vi "RemoteVI Loop Flags.vi"(0 "clients":T1(array[cluster]), 5 "last geometry":u32, 7 "last click":u32, 9 "popup was open?":bool) -> (4 "now":u32, 6 "look?":bool, 8 "geometry due?":bool, 10 "remote click?":bool, 15 "recent click?":bool)   [LabVIEW 2020, in "RemoteVI.lvlib"]
doc: "The timing decisions at the start of a server loop iteration: now (tick count ms); geometry due? when 500 ms have passed since last geometry; look? (list the popups) when a client is connected, the geometry is due or a popup was open last time; remote click? within 1 s and recent click? within 300 ms after a client last posted a message that may open a popup (last click). Pure apart from reading the tick count."
uses:
  RemoteVI.lvlib
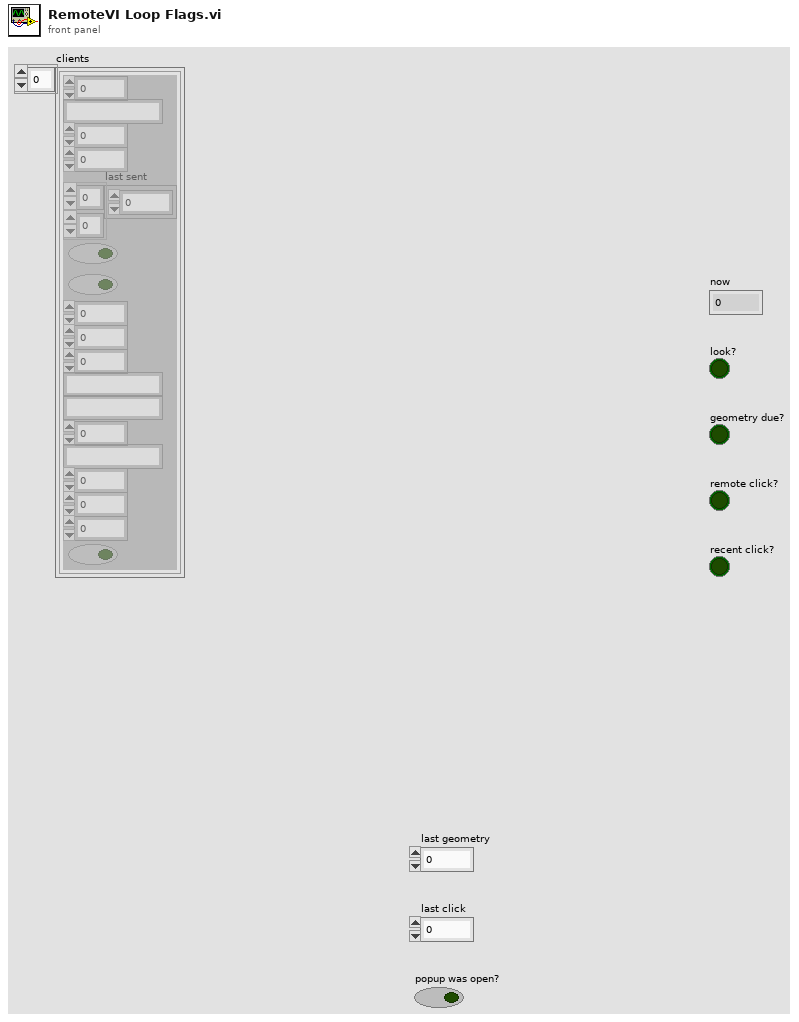
[diagram p1: front panel]
types:
  T1 = cluster{"connection":u32, "rx buffer":string, "seq":u32, "acked":u32, "last sent":u32[][], "tracking":bool, "closed":bool, "mods":u8, "mods set":u8, "popup since":u32, "windows sent":string, "window frames":cluster{"id":u64, "pixels":u32[][]}[], "key window":u64, "address":string, "since":dbl, "last input":dbl, "bytes":dbl, "view only":bool}[]
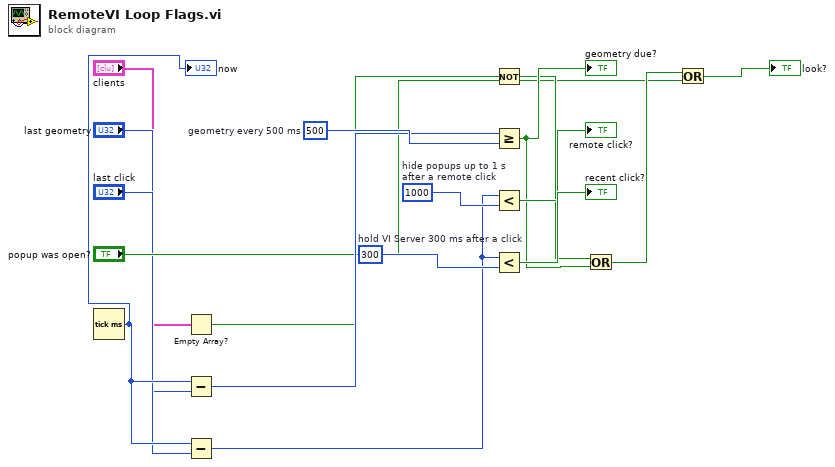
[diagram p0: block diagram]
diagram:
  w16 = u32 300  # hold VI Server 300 ms after a click
  w14 = u32 1000  # hide popups up to 1 s after a remote click
  w9 = u32 500  # geometry every 500 ms
  n1 = Tick Count (ms)() -> (millisecond timer value=w5:u32)
  "now" <- w5
  n2 = Empty Array?(array="clients") -> (empty?=w6:bool)
  n3 = Subtract(x=w5, y="last geometry") -> (x-y=w8:u32)
  n4 = Subtract(x=w5, y="last click") -> (x-y=w13:u32)
  n5 = Not(x=w6) -> (.not. x?=w7:bool)
  n6 = Greater Or Equal?(x=w8, y=w9) -> (x >= y?=w10:bool)
  "geometry due?" <- w10
  n7 = Less?(x=w13, y=w14) -> (x < y?=→"remote click?":bool)
  n8 = Less?(x=w13, y=w16) -> (x < y?=→"recent click?":bool)
  n9 = Or(x=w7, y=w10) -> (x .or. y?=w11:bool)
  n10 = Or(x=w11, y="popup was open?") -> (x .or. y?=→"look?":bool)
